vi "Smart IO Get Digital Input.vi"(6 "force":bool, 8 "error in (no error)":errorcluster, 11 "deviceIndex":i32) -> (0 "error out":errorcluster, 2 "value out":bool)   [LabVIEW 2023, in "MrcLib.lvlib"]
doc: "Return the instantaneous state of the digital I/O pin for the indicated device channel. Logical TRUE means signal is ???"
uses:
  <vilib>/MRC/MrcLib.lvlib
  <vilib>/MRC/Types/MRC Smart IO Mode.ctl
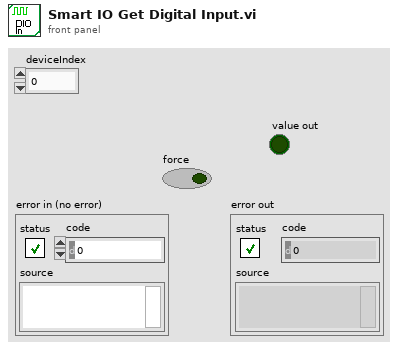
[diagram p1: front panel]
types:
  T1 = typedef "MRC Smart IO Mode.ctl" = i32
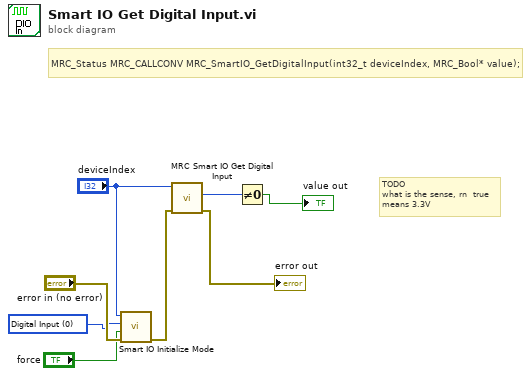
[diagram p0: block diagram]
diagram:
  w2 = T1 0 items=["Digital Input"=0, "Digital Output"=1, "Analog Input"=2, "PWM Input"=3, "PWM Output"=4, "Counter Rising"=5, "Counter Falling"=6, "Addressable LEDs"=13] ("mode")
  # "TODO\nwhat is the sense, rn  true\nmeans 3.3V"
  # "MRC_Status MRC_CALLCONV MRC_SmartIO_GetDigitalInput(int32_t deviceIndex, MRC_Bool* value);"
  n1 = call <vilib>:"Smart IO Initialize Mode.vi"("error in (no error)"="error in (no error)", "force"="force", "mode"=w2, "deviceIndex"="deviceIndex") -> ("error out"=w4:errorcluster)  [unwired: 7 in]
  n2 = call <vilib>:"MRC Smart IO Get Digital Input.vi"("error in (no error)"=w4, "deviceIndex"="deviceIndex") -> ("error out"=→"error out":errorcluster, "value out"=w7:u8)  [unwired: 8 in]
  n3 = Not Equal To 0?(x=w7) -> (x != 0?=→"value out":bool)
